vi "Sync.Destroy.vi"(8 "error in (no error)":errorcluster, 11 "DAQmx in":refnum<class "DAQmx.lvclass">) -> (0 "error out":errorcluster, 3 "DAQmx out":refnum<class "DAQmx.lvclass">)   [LabVIEW 2019, in "DAQmx.lvclass"]
uses:
  DAQmx.lvclass
  DAQmx.lvclass/DAQmx.ctl
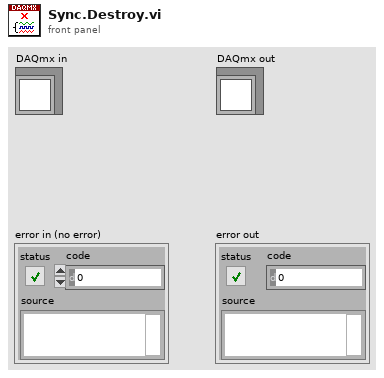
[diagram p1: front panel]
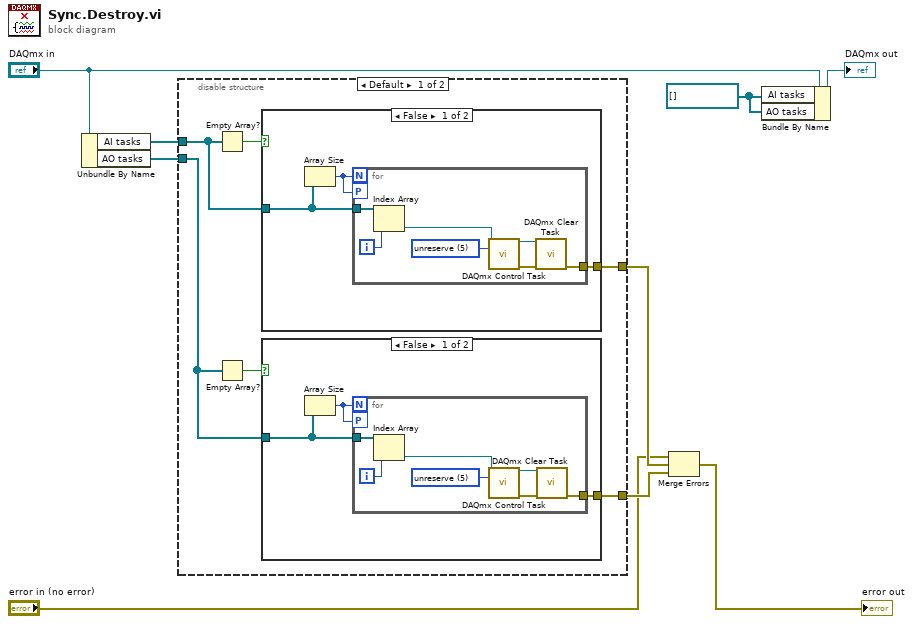
[diagram p0: block diagram]
diagram:
  w1 = refnum<k21>[] [] ("AI task")
  n1 = Unbundle By Name("DAQmx in") -> ("AI tasks"=w8:refnum<k21>[], "AO tasks"=w9:refnum<k21>[])
  n2 = disable-structure shown="Default" {
    disable-tunnel: [w15 _] -> w4
    disable-tunnel: w9 -> [w12 _]
    disable-tunnel: w8 -> [w13 _]
    disable-tunnel: [w11 _] -> w5
    frame condition #0 (active) {
      n3 = Empty Array?(array=w13) -> (empty?=w14:bool)
      n4 = Empty Array?(array=w12) -> (empty?=w10:bool)
      n5 = case shown="False" w14 {
        tunnel: w13 -> [w27 _]
        tunnel: [w28 _] -> w15
        frame False {
          n6 = Array Size(array=w27) -> (size(s)=w26:i32)
          n7 = for {
            N: w26 -> [_]
            tunnel: w27 -> [w34]
            tunnel: [w30] -> w28
            workers-P: w26 -> [_]
            i -> [w35]
            w33 = 5 items=["verify"=2, "reserve"=4, "commit"=3, "unreserve"=5, "abort"=6] ("action")
            n8 = Index Array(array=w34, index=w35) -> (element=w32:refnum<k21>)
            n9 = call <vilib>:"DAQmx Control Task.vi"("task/channels in"=w32, "action"=w33) -> ("task out"=w29:refnum<k21>, "error out"=w31:errorcluster)  [unwired: 12 in]
            n10 = call <vilib>:"DAQmx Clear Task.vi"("task in"=w29, "error in"=w31) -> ("error out"=w30:errorcluster)  [unwired: 13 in]
          }
        }
        frame True {
        }
      }
      n11 = case shown="False" w10 {
        tunnel: w12 -> [w17 _]
        tunnel: [w18 _] -> w11
        frame False {
          n12 = Array Size(array=w17) -> (size(s)=w16:i32)
          n13 = for {
            N: w16 -> [_]
            tunnel: w17 -> [w24]
            tunnel: [w19] -> w18
            workers-P: w16 -> [_]
            i -> [w25]
            w23 = 5 items=["verify"=2, "reserve"=4, "commit"=3, "unreserve"=5, "abort"=6] ("action")
            n14 = Index Array(array=w24, index=w25) -> (element=w22:refnum<k21>)
            n15 = call <vilib>:"DAQmx Control Task.vi"("task/channels in"=w22, "action"=w23) -> ("task out"=w21:refnum<k21>, "error out"=w20:errorcluster)  [unwired: 12 in]
            n16 = call <vilib>:"DAQmx Clear Task.vi"("task in"=w21, "error in"=w20) -> ("error out"=w19:errorcluster)  [unwired: 13 in]
          }
        }
        frame True {
        }
      }
    }
    frame condition #1 {
    }
  }
  n17 = Merge Errors("error in (no error)", w4, w5) -> (→"error out":errorcluster)
  n18 = Bundle By Name(cluster="DAQmx in", "AI tasks"=w1, "AO tasks"=w1) -> (→"DAQmx out":refnum<class "DAQmx.lvclass">)
